vi "Handle Value Change.vi"(5 "VolatusAPI":refnum<class "VolatusAPI.lvclass">, 7 "CtlRef":refnum<vi>, 8 "error in (no error)":errorcluster, 9 "NewVal":variant, 10 "OldVal":variant, 11 "NumericCommandButton in":refnum<class "NumericCommandButton.lvclass">) -> (0 "error out":errorcluster, 3 "NumericCommandButton out":refnum<class "NumericCommandButton.lvclass">)   [LabVIEW 2025, in "VolatusGUIElements.lvlib" / "NumericCommandButton.lvclass"]
uses:
  NumericCommandButton.lvclass
  Volatus/VolatusAPI/VolatusAPI.lvclass
  NumericCommandButton.lvclass/NumericCommandButton.ctl
  C:/dev/volatus/mts-volatus-super/libs/lv-volatus/VolatusGUI/GUI Element/GUI Element.lvclass
  C:/dev/volatus/mts-volatus-super/libs/lv-volatus/VolatusGUIElements/NumericCommandButton/NumericCommandButton.lvclass
  C:/dev/volatus/mts-volatus-super/libs/lv-volatus/VolatusGUI/OnValueChangeHandler/OnValueChangeHandler.lvclass
  Volatus/Numeric Command/Numeric Command.lvclass
  VolatusGUI/GUI Element/GUI Element.lvclass
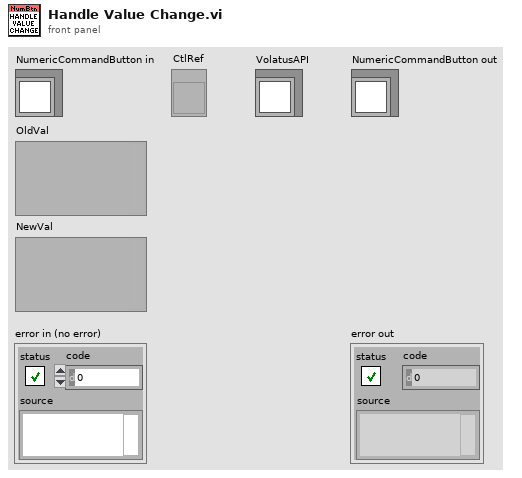
[diagram p1: front panel]
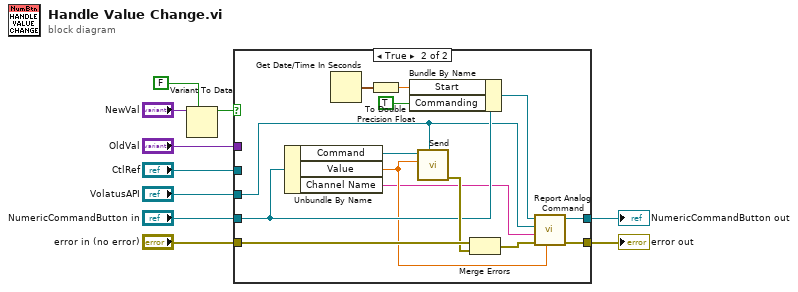
[diagram p0: block diagram]
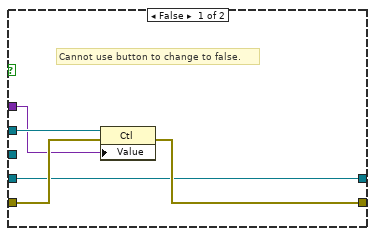
[diagram p2: hidden frame]
diagram:
  n1 = Variant To Data(type=FALSE, Variant="NewVal") -> (data=w8:bool)  [unwired: 1 in, 1 out]
  n2 = case shown="True" w8 {
    tunnel: "OldVal" -> [w11 _]
    tunnel: "CtlRef" -> [w12 _]
    tunnel: "error in (no error)" -> [w14 w28]
    tunnel: [w13 w22] -> w4
    tunnel: "NumericCommandButton in" -> [w13 w26]
    tunnel: [w15 w19] -> w2
    tunnel: "VolatusAPI" -> [_ w18]
    frame False {
      # "Cannot use button to change to false."
      n3 = property class="Ctl"(reference=w12, error in=w14, "Value"=w11) -> (error out=w15:errorcluster)  [unwired: 1 out]
    }
    frame True {
      n4 = Unbundle By Name(w26) -> ("Command"=w29:refnum<class "Numeric Command.lvclass">, "Value"=w17:dbl, "Channel Name"=w16:string)
      n5 = Get Date/Time In Seconds() -> (seconds since 1Jan1904=w24:timestamp)
      n6 = To Double Precision Float(number=w24) -> (double precision float=w23:dbl)
      n7 = Bundle By Name(cluster=w26, "Start"=w23, "Commanding"=TRUE) -> (w21:refnum<class "NumericCommandButton.lvclass">)
      n8 = call "Send.vi"("VolatusAPI"=w18, "Value"=w17, "Numeric Command in"=w29) -> ("error out"=w27:errorcluster)  [unwired: 8 in]
      n9 = Merge Errors(w28, w27) -> (w20:errorcluster)
      n10 = call "Report Analog Command.vi"("Value"=w17, "error in (no error)"=w20, "Name"=w16, "VolatusAPI in"=w18, "GUI Element in"=w21) -> ("error out"=w19:errorcluster, "GUI Element out"=w22:refnum<class "NumericCommandButton.lvclass">)  [unwired: 5 in]
    }
  }
  "error out" <- w2
  "NumericCommandButton out" <- w4
